vi "UnlinkNode.vi"(8 "error in":errorcluster, 10 "child in":T1, 11 "parent in":T1) -> (0 "error out":errorcluster, 2 "child out":T1, 3 "parent out":T1)   [LabVIEW 2014, in "NISE_CEF_Node.lvclass"]
doc: "Breaks the link between a child and a parent node. Removing the reference to each other in both nodes."
uses:
  NISE_CEF_Node.lvclass
  NodeRef.ctl
  NISE_CEF_Node.lvclass/NISE_CEF_Node.ctl
  ReadChildren.vi
  WriteParent.vi
  WriteChildren.vi
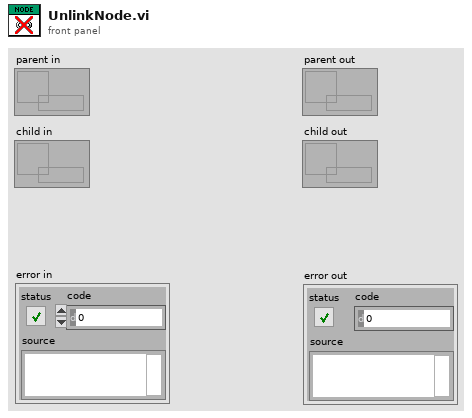
[diagram p1: front panel]
types:
  T1 = typedef "NISE_CEF_Node.lvclass/NodeRef.ctl" = refnum<data-value>
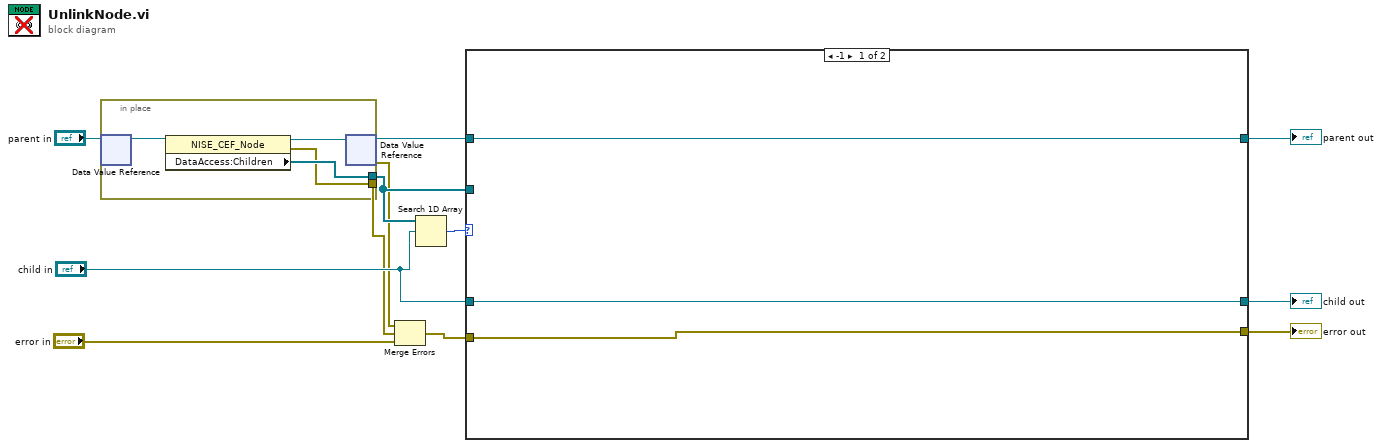
[diagram p0: block diagram]
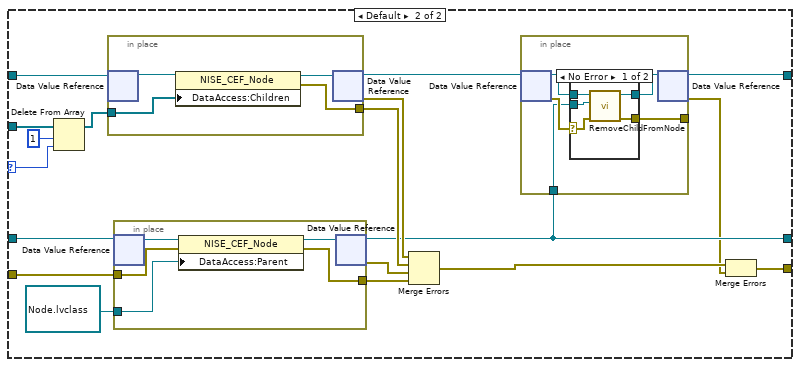
[diagram p2: hidden frame]
diagram:
  n1 = in-place {
    in-place-border: [w14] -> w10
    in-place-border: [w13] -> w2
    n2 = in-place-dvr #1("parent in") -> (w16:refnum<class "NISE_CEF_Node.lvclass">)  [unwired: 1 out]
    n3 = property class="NISE_CEF_Node"(reference=w16) -> (reference out=w15:refnum<class "NISE_CEF_Node.lvclass">, error out=w13:errorcluster, "DataAccess:Children"=w14:T1[])  [unwired: 1 in]
    n4 = in-place-dvr #1(w15) -> (w11:T1, w1:errorcluster)
  }
  n5 = Merge Errors(w1, w2, "error in") -> (w3:errorcluster)
  n6 = Search 1D Array(1D array=w10, element="child in") -> (index of element=w12:i32)  [unwired: 1 in]
  n7 = case shown="-1" w12 {
    selector: w12 -> [_ w33]
    tunnel: "child in" -> [w17 w37]
    tunnel: w3 -> [w19 w36]
    tunnel: [w19 w22] -> w9
    tunnel: w11 -> [w18 w31]
    tunnel: [w18 w24] -> w5
    tunnel: [w17 w23] -> w6
    tunnel: w10 -> [_ w35]
    frame -1 {
    }
    frame Default {
      n8 = Delete From Array(array=w35, length=1, index=w33) -> (array with subset deleted=w32:T1[])  [unwired: 1 out]
      n9 = in-place {
        in-place-border: w32 -> [w51]
        in-place-border: [w50] -> w29
        n10 = in-place-dvr #2(w31) -> (w53:refnum<class "NISE_CEF_Node.lvclass">)  [unwired: 1 out]
        n11 = property class="NISE_CEF_Node"(reference=w53, "DataAccess:Children"=w51) -> (reference out=w52:refnum<class "NISE_CEF_Node.lvclass">, error out=w50:errorcluster)  [unwired: 1 in]
        n12 = in-place-dvr #2(w52) -> (w25:T1, w28:errorcluster)
      }
      n13 = in-place {
        in-place-border: w36 -> [w57]
        in-place-border: refnum<data-value> refnum ("parent out") -> [w55]
        in-place-border: [w54] -> w27
        n14 = in-place-dvr #3(w37) -> (w58:refnum<class "NISE_CEF_Node.lvclass">)  [unwired: 1 out]
        n15 = property class="NISE_CEF_Node"(reference=w58, error in=w57, "DataAccess:Parent"=w55) -> (reference out=w56:refnum<class "NISE_CEF_Node.lvclass">, error out=w54:errorcluster)
        n16 = in-place-dvr #3(w56) -> (w23:T1, w26:errorcluster)
      }
      n17 = Merge Errors(w28, w29, w26, w27) -> (w21:errorcluster)
      n18 = in-place {
        in-place-border: [w42] -> _
        in-place-border: w23 -> [w38]
        n19 = in-place-dvr #4(w25) -> (w41:refnum<class "NISE_CEF_Node.lvclass">, w39:errorcluster)
        n20 = case shown="No Error" w39 {
          selector: w39 -> [w43 w48]
          tunnel: [w47 w48] -> w42
          tunnel: w41 -> [w46 w49]
          tunnel: [w45 w49] -> w40
          tunnel: w38 -> [w44 _]
          frame No Error {
            n21 = call-dynamic "RemoveChildFromNode.vi"("error in"=w43, "removed child"=w44, "NISE_CEF_Node in"=w46) -> ("error out"=w47:errorcluster, "NISE_CEF_Node out"=w45:refnum<class "NISE_CEF_Node.lvclass">)  [unwired: 7 in]
          }
          frame Error {
          }
        }
        n22 = in-place-dvr #4(w40) -> (w24:T1, w20:errorcluster)
      }
      n23 = Merge Errors(w21, w20) -> (w22:errorcluster)
    }
  }
  "child out" <- w6
  "parent out" <- w5
  "error out" <- w9
